vi "Functional Test.vi"() -> ()   [LabVIEW 2018]
uses:
  src/api/logger_class/Failure Information.ctl
  src/api/logger_class/Log Record.ctl
  src/api/logger_class/Internal Log Levels.ctl
  3ae5ef6d-8e83-4c37-89d5-c4af1027e008.vi
  d7f581ef-27d1-4084-8bbe-9e7418d10964.vi
  d7f581ef-27d1-4084-8bbe-9e7418d10964.vi/caf2d4a3-5a7b-40e1-b7b0-74b52901b9f9.vi
  d7f581ef-27d1-4084-8bbe-9e7418d10964.vi/caf2d4a3-5a7b-40e1-b7b0-74b52901b9f9.vi/0a1ee2ab-da6d-4243-8cf3-8125e611a602.vi
  src/api/Log.vi
  src/api/configuration/formatters/format_string_formatter/Format String.lvclass
  C:/Users/Colin/Documents/software_projects/labview/glog/src/api/extension/formatter_interface/Formatter.lvclass
  src/api/configuration/handlers/string_handler/String Handler.lvclass
  C:/Users/Colin/Documents/software_projects/labview/glog/src/api/extension/formatting_handler_interface/Formatting Handler.lvclass
  src/registry/Log.vi
  src/api/GLog.lvlib
  src/api/logger_class/Logger.lvclass
panel:
  in  "log count limit (500)":u32=500
  in  "line count limit (500)":u32=500
  in  "loop delay [ms]":u32
  in  "iterations":i32=20
  out "failures info":T1[](array[typedef]) {"Log Record"."timestamp" format="%<%x %.3X>T"}
  out "error out":errorcluster
  in  "multi-line w/auto-scroll":string
  in  "single line":string
  in  "multi-line":string
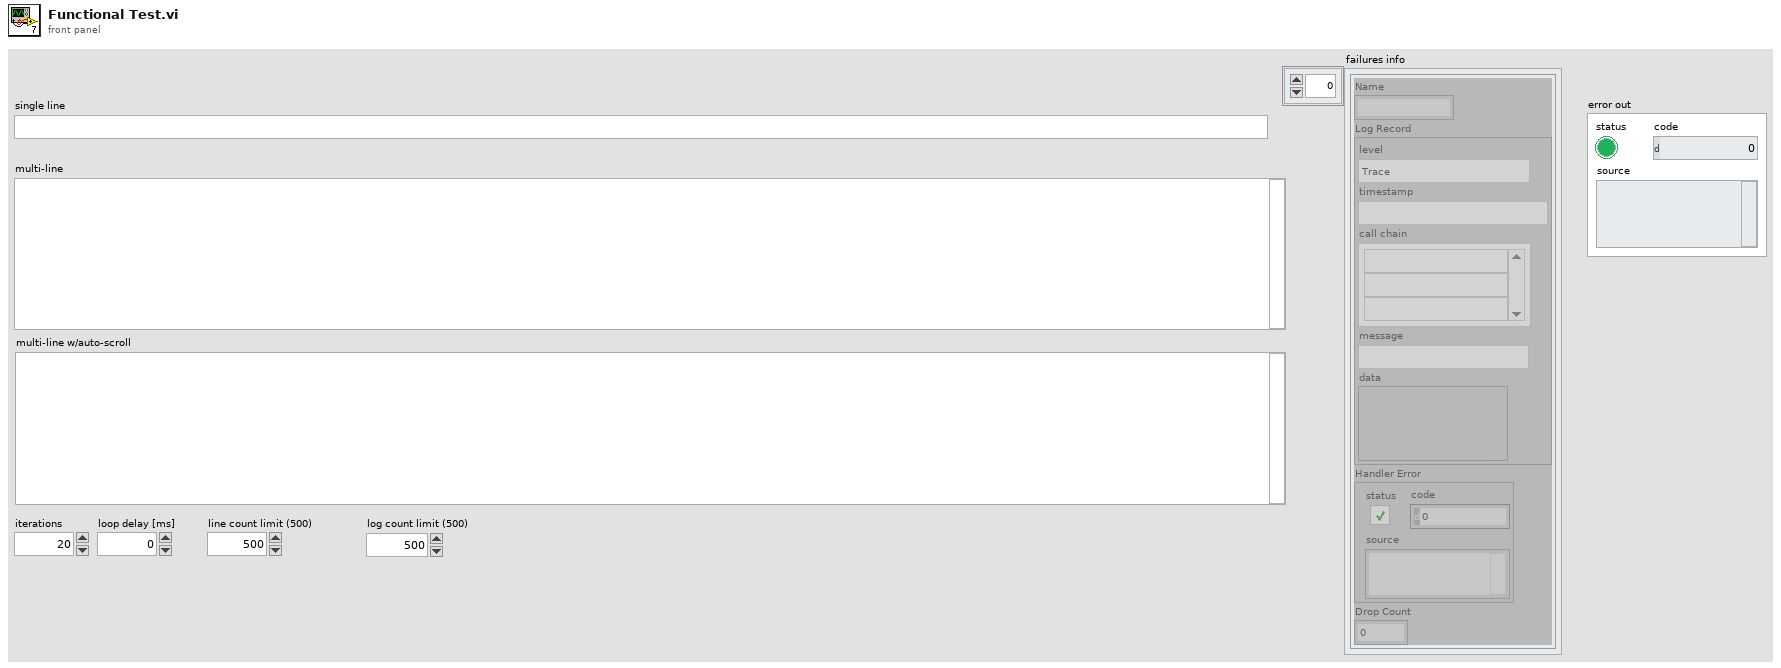
[diagram p1: front panel]
types:
  T1 = typedef "GLog.lvlib/Logger.lvclass/Failure Information.ctl" = cluster{"Name":string, "Log Record":T2, "Handler Error":errorcluster, "Drop Count":u32}
  T2 = typedef "GLog.lvlib/Logger.lvclass/Log Record.ctl" = cluster{"level":T3, "timestamp":timestamp, "call chain":string[], "message":string, "data":variant}
  T3 = typedef "GLog.lvlib/Logger.lvclass/Internal Log Levels.ctl" = enum16{"Trace", "Debug", "Info", "Warning", "Error", "Critical", "Internal"}
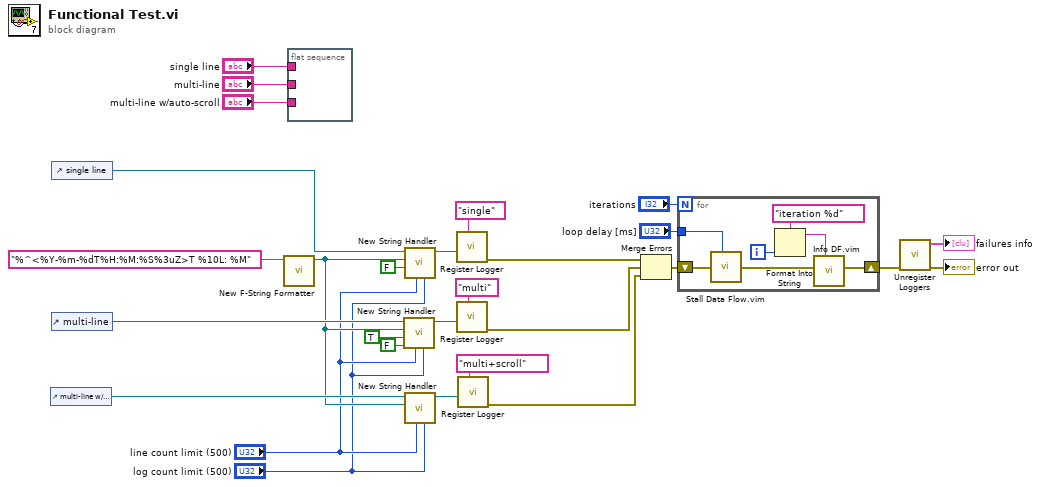
[diagram p0: block diagram]
diagram:
  n1 = control-ref of="multi-line w/auto-scroll"() -> (w26:refnum<vi>)
  n2 = control-ref of="single line"() -> (w28:refnum<vi>)
  n3 = control-ref of="multi-line"() -> (w27:refnum<vi>)
  n4 = call "New F-String Formatter.vi"("format string (\"%T | %L | %M\")"="%^<%Y-%m-%dT%H:%M:%S%3uZ>T %10L: %M" ("format string")) -> ("new f-string formatter"=w10:refnum<class "Format String.lvclass">)  [unwired: 10 in]
  n5 = flat-sequence {
    tunnel: "single line" -> [_]
    tunnel: "multi-line" -> [_]
    tunnel: "multi-line w/auto-scroll" -> [_]
    frame #0 {
    }
  }
  n6 = call "New String Handler.vi"("log count limit (500)"="log count limit (500)", "line count limit (500)"="line count limit (500)", "auto-scroll? (T)"=FALSE, "multi-line? (T)"=TRUE, "formatter (format string)"=w10, "string control"=w27) -> ("new string handler"=w4:refnum<class "String Handler.lvclass">)  [unwired: 5 in]
  n7 = call "New String Handler.vi"("log count limit (500)"="log count limit (500)", "line count limit (500)"="line count limit (500)", "multi-line? (T)"=FALSE, "formatter (format string)"=w10, "string control"=w28) -> ("new string handler"=w6:refnum<class "String Handler.lvclass">)  [unwired: 6 in]
  n8 = call "New String Handler.vi"("log count limit (500)"="log count limit (500)", "line count limit (500)"="line count limit (500)", "formatter (format string)"=w10, "string control"=w26) -> ("new string handler"=w24:refnum<class "String Handler.lvclass">)  [unwired: 7 in]
  n9 = call "Register Logger.vi"("name (\"Default\")"="single" ("name (\"Default\")"), "log handler (file handler)"=w6) -> ("error out"=w23:errorcluster)  [unwired: 9 in]
  n10 = call "Register Logger.vi"("name (\"Default\")"="multi" ("name (\"Default\")"), "log handler (file handler)"=w4) -> ("error out"=w22:errorcluster)  [unwired: 9 in]
  n11 = call "Register Logger.vi"("name (\"Default\")"="multi+scroll" ("name (\"Default\")"), "log handler (file handler)"=w24) -> ("error out"=w21:errorcluster)  [unwired: 9 in]
  n12 = Merge Errors(w23, w22, w21) -> (w20:errorcluster)
  n13 = for {
    N: "iterations" -> [_]
    shift-right: [w31] -> w11
    shift-left: w20 -> [w35]
    tunnel: "loop delay [ms]" -> [w29]
    i -> [w34]
    n14 = call "Stall Data Flow.vim"("value in"=w35, "milliseconds to wait"=w29) -> ("value out"=w30:errorcluster)  [unwired: 1 out]
    n15 = Format Into String(format string="iteration %d", w34) -> (resulting string=w32:string)  [unwired: 2 in, 1 out]
    n16 = call "Info DF.vim"("message"=w32, "dataflow in"=w30) -> ("dataflow out"=w31:errorcluster)  [unwired: 9 in]
  }
  n17 = call "Unregister Loggers.vi"("error in (no error)"=w11) -> ("error out"=→"error out":errorcluster, "failures info"=→"failures info":T1[])  [unwired: 9 in]
